vi "Calculate PWM Range&Data.vi"(8 "error in (no error)":errorcluster, 9 "Duty Cycle":dbl=0.5, 10 "PWM Freq":dbl=100.0, 11 "PWM Clock Divider":i32) -> (0 "error out":errorcluster, 1 "Actual Duty Cycle":dbl=100.0, 2 "Actual Freq":dbl=100.0, 3 "PWM Range":i32, 5 "PWM Data":i32)   [LabVIEW 2020, in "wiringPi.lvlib"]
doc: "<<b>_______________________________________________________________</b>\n** Author: Juan José Villacorta\n** LabVIEW wrapper for C library <b> wiringPi </b>,\n** https://github.com/WiringPi/WiringPi\n<b>_______________________________________________________________</b>\n\nSet the PWM frequency and duty-cycle\nCalculate a PWM 'range' and 'value' setting using the PWM Clock Divider and desired PWM frecuency. Uses the formula: range (u32) = (19.2 MHz )/Divider/Frecuency"
uses:
  wiringPi.lvlib
  <vilib>/ErrorRing/Error Ring.xnode
  <vilib>/Utility/error.llb/Error Cluster From Error Code.vi
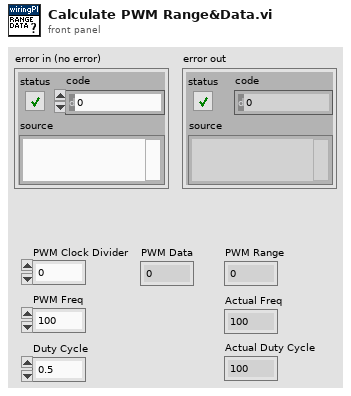
[diagram p1: front panel]
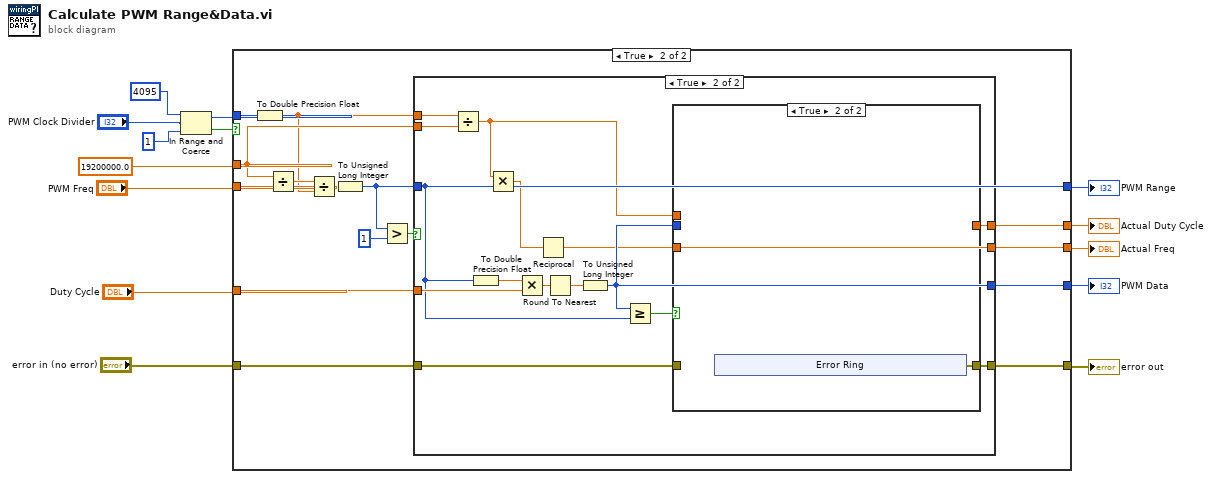
[diagram p0: block diagram]
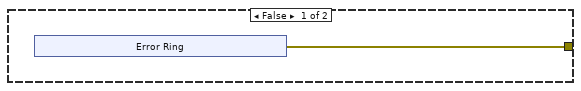
[diagram p2: hidden frame]
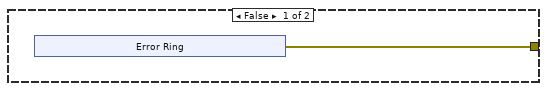
[diagram p3: hidden frame]
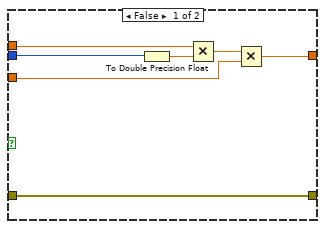
[diagram p4: hidden frame]
diagram:
  n1 = In Range and Coerce(upper limit=4095, x="PWM Clock Divider", lower limit=1) -> (coerced(x)=w6:i32, In Range?=w5:bool)
  n2 = case shown="True" w5 {
    tunnel: "PWM Freq" -> [_ w35]
    tunnel: w6 -> [_ w32]
    tunnel: "Duty Cycle" -> [_ w31]
    tunnel: 19200000.0 ("x") -> [_ w28]
    tunnel: [_ w22] -> w11
    tunnel: [_ w30] -> w10
    tunnel: "error in (no error)" -> [_ w21]
    tunnel: [w15 w23] -> w3
    tunnel: [_ w25] -> w2
    tunnel: [_ w29] -> w1
    frame False {
      n3 = xnode "Error Ring"() -> ("error out"=w15:errorcluster)
    }
    frame True {
      n4 = To Double Precision Float(number=w32) -> (double precision float=w27:dbl)
      n5 = Divide(x=w28, y=w35) -> (x/y=w34:dbl)
      n6 = Divide(x=w34, y=w27) -> (x/y=w33:dbl)
      n7 = To Unsigned Long Integer(number=w33) -> (unsigned 32bit integer=w25:u32)
      n8 = Greater?(x=w25, y=u32 1) -> (0:w26:bool)
      n9 = case shown="True" w26 {
        tunnel: w31 -> [_ w54]
        tunnel: [_ w42] -> w30
        tunnel: w25 -> [_ w46]
        tunnel: [_ w47] -> w29
        tunnel: w28 -> [_ w51]
        tunnel: w27 -> [_ w50]
        tunnel: [w36 w45] -> w23
        tunnel: [_ w48] -> w22
        tunnel: w21 -> [_ w44]
        frame False {
          n10 = xnode "Error Ring"() -> ("error out"=w36:errorcluster)
        }
        frame True {
          n11 = Divide(x=w50, y=w51) -> (x/y=w49:dbl)
          n12 = To Double Precision Float(number=w46) -> (double precision float=w56:dbl)
          n13 = Multiply(x=w49, y=w46) -> (x*y=w52:dbl)
          n14 = Multiply(x=w56, y=w54) -> (x*y=w55:dbl)
          n15 = Reciprocal(x=w52) -> (1/x=w42:dbl)
          n16 = Round To Nearest(number=w55) -> (nearest integer value=w53:dbl)
          n17 = To Unsigned Long Integer(number=w53) -> (unsigned 32bit integer=w47:u32)
          n18 = Greater Or Equal?(x=w47, y=w46) -> (x >= y?=w43:bool)
          n19 = case shown="True" w43 {
            tunnel: w42 -> [w59 _]
            tunnel: w49 -> [w60 _]
            tunnel: [w58 _] -> w48
            tunnel: w47 -> [w57 _]
            tunnel: [w63 w64] -> w45
            tunnel: w44 -> [w63 _]
            frame False {
              n20 = To Double Precision Float(number=w57) -> (double precision float=w61:dbl)
              n21 = Multiply(x=w60, y=w61) -> (x*y=w62:dbl)
              n22 = Multiply(x=w62, y=w59) -> (x*y=w58:dbl)
            }
            frame True {
              n23 = xnode "Error Ring"() -> ("error out"=w64:errorcluster)
            }
          }
        }
      }
    }
  }
  "Actual Freq" <- w10
  "Actual Duty Cycle" <- w11
  "error out" <- w3
  "PWM Range" <- w2
  "PWM Data" <- w1
